vi "VIH Project Tree - Find Group to Add Item.vi"(8 "error in":errorcluster, 10 "Item Tag":string, 11 "Project Tree":T1) -> (0 "error out":errorcluster, 2 "Item Tag (Group)":string, 3 "dup Project Tree":T1)   [LabVIEW 2014]
doc: "::: VI Helpeks :::\nCopyright (c) 2000-2026 Konstantin Shifershteyn. All rights reserved."
uses:
  VIH Project Tree Typedef - Tree Refnum.ctl
  VIH Project Tree Typedef - Tree Item Type.ctl
panel:
  # "VI Helpeks\nCopyright (c) 2012-2026 Konstantin Shifershteyn"
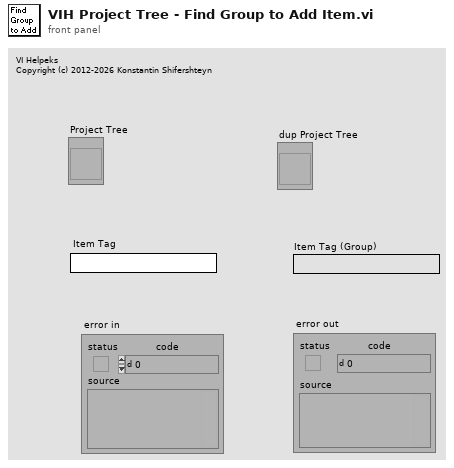
[diagram p1: front panel]
types:
  T1 = typedef "VIH Project Tree Typedef - Tree Refnum.ctl" = refnum<vi>
  T2 = typedef "VIH Project Tree Typedef - Tree Item Type.ctl" = enum32{"<Invalid>", "Project", "Proj Files", "Proj Rules", "File Group", "Rule Group", "Any File", "LV Func", ".mnu", ".mnu (dyn)", ".vi", ".vi (dyn)", ".vit", ".vit (dyn)", ".ctl", ".ctl (dyn)", ".ctt", ".ctt (dyn)", "polyVI", "polyVI (dyn)", "expVI", "expVI (dyn)", "HTML", "PolyVI Inst"}
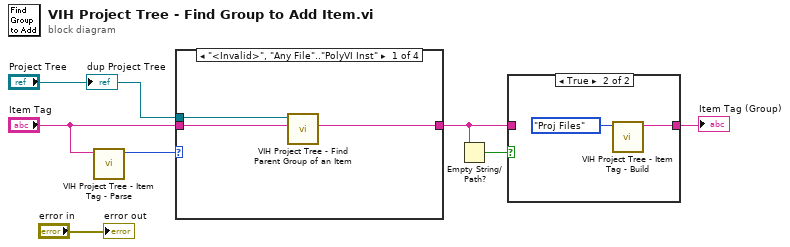
[diagram p0: block diagram]
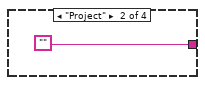
[diagram p3: hidden frame]
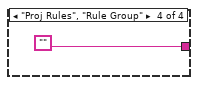
[diagram p5: hidden frame]
diagram:
  n1 = call "VIH Project Tree - Item Tag - Parse.vi"("Tree Item Tag"="Item Tag") -> ("Item Type"=w7:T2)  [unwired: 8 in, 2 out]
  n2 = case shown="\"<Invalid>\", \"Any File\"..\"PolyVI Inst\"" w7 {
    tunnel: [w10 "" w12 ""] -> w3
    tunnel: "Item Tag" -> [w9 _ w12 _]
    tunnel: "Project Tree" -> [w8 _ _ _]
    frame "<Invalid>", "Any File".."PolyVI Inst" {
      n3 = call "VIH Project Tree - Find Parent Group of an Item.vi"("Tree Item Tag"=w9, "Project Tree"=w8) -> ("Parent Group Tag"=w10:string)  [unwired: 6 in, 3 out]
    }
    frame "Project" {
    }
    frame "Proj Files", "File Group" {
    }
    frame "Proj Rules", "Rule Group" {
    }
  }
  n4 = Empty String/Path?(string/path=w3) -> (empty?=w4:bool)
  n5 = case shown="True" w4 {
    tunnel: [w14 w15] -> w5
    tunnel: w3 -> [w14 _]
    frame False {
    }
    frame True {
      n6 = call "VIH Project Tree - Item Tag - Build.vi"("Item Type"=VIH_Project_Tree_Typedef_-_Tree_Item_Type."Proj Files") -> ("Tree Item Tag"=w15:string)  [unwired: 9 in, 1 out]
    }
  }
  "Item Tag (Group)" <- w5
  "error out" <- "error in"
  "dup Project Tree" <- "Project Tree"
